vi "OwnCompat20261012_Native_Wire.vi"() -> ()   [LabVIEW 2024]
panel:
  out "error out":errorcluster caption="错误输出"
  in  "sink_terminal":u32
  in  "source_terminal":u32
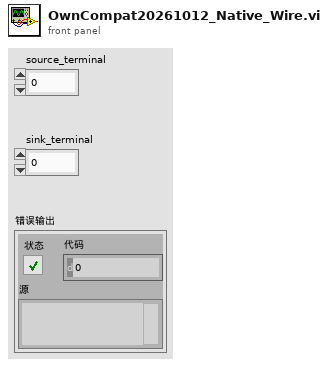
[diagram p1: front panel]
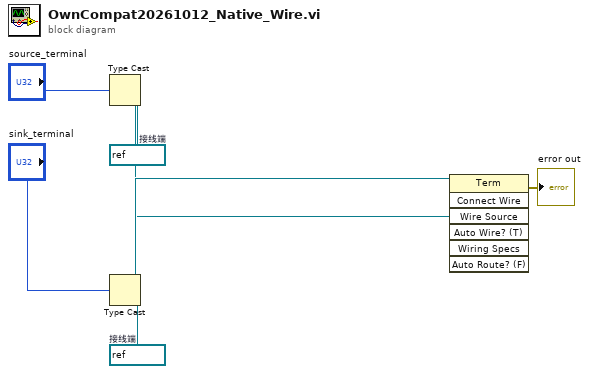
[diagram p0: block diagram]
diagram:
  w4 = refnum<vi> refnum  # 接线端
  w6 = refnum<vi> refnum  # 接线端
  n1 = Type Cast ("强制类型转换")(type=w6, x="source_terminal") -> (*(type *) &x=w2:refnum<vi>)
  n2 = Type Cast ("强制类型转换")(type=w4, x="sink_terminal") -> (*(type *) &x=w3:refnum<vi>)
  n3 = invoke class="Term" method="Connect Wire"(reference=w3, "Wire Source"=w2) -> (error out=→"error out":errorcluster)  [unwired: 5 in, 6 out]
